vi "async stream processor.vi"(8 "error return queue":refnum<queue>, 9 "dataset RID":string, 10 "api key":string, 11 "data queue":refnum<queue>) -> (0 "last error":errorcluster)   [LabVIEW 2020, in "Nominal-Streamer.lvlib" / "Nominal-Streamer.lvclass"]
uses:
  Nominal-Streamer.lvclass
  <vilib>/Nominal/Nominal IO Client/submodules/nominal-streaming-labview-ffi/lv_src/Channel/Channel.lvclass
  <vilib>/Nominal/Nominal IO Client/lv_src/Nominal Client/Nominal Client.lvclass/Nominal Client.ctl
  <vilib>/Nominal/Nominal IO Client/lv_src/User/User.lvclass
  <vilib>/Nominal/Nominal IO Client/lv_src/Nominal Client/Nominal Client.lvclass
  <vilib>/Nominal/Nominal IO Client/lv_src/nominal types/workspace/workspace.lvclass
  <vilib>/Nominal/Nominal IO Client/submodules/reqwest-labview/lv-src/reqwest/reqwest.lvclass
  Nominal-Streamer.lvclass/Nominal-Streamer.ctl
  86105a90-7170-41be-9865-40c2d640c79f.vi
  <vilib>/Nominal/Nominal IO Client/submodules/nominal-streaming-labview-ffi/lv_src/Stream/Stream.lvclass
  <vilib>/Nominal/Nominal IO Client/lv_src/datasources/dataset/dataset.lvclass
  <vilib>/Utility/miscctls.llb/LVMapReplaceAction.ctl
  <vilib>/Utility/SystemLogging/NI_SystemLogging.lvlib
  async queue data.ctl
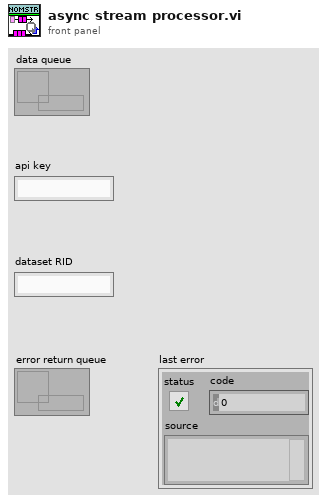
[diagram p1: front panel]
types:
  T1 = typedef "LVMapReplaceAction.ctl" = enum32{"Modify Entry only if found", "Add or Modify Entry", "Delete Entry"}
  T2 = typedef "Nominal-Streamer.lvlib/Nominal-Streamer.lvclass/async queue data.ctl" = cluster{"data values":waveform(dbl)[], "data names":string[]}
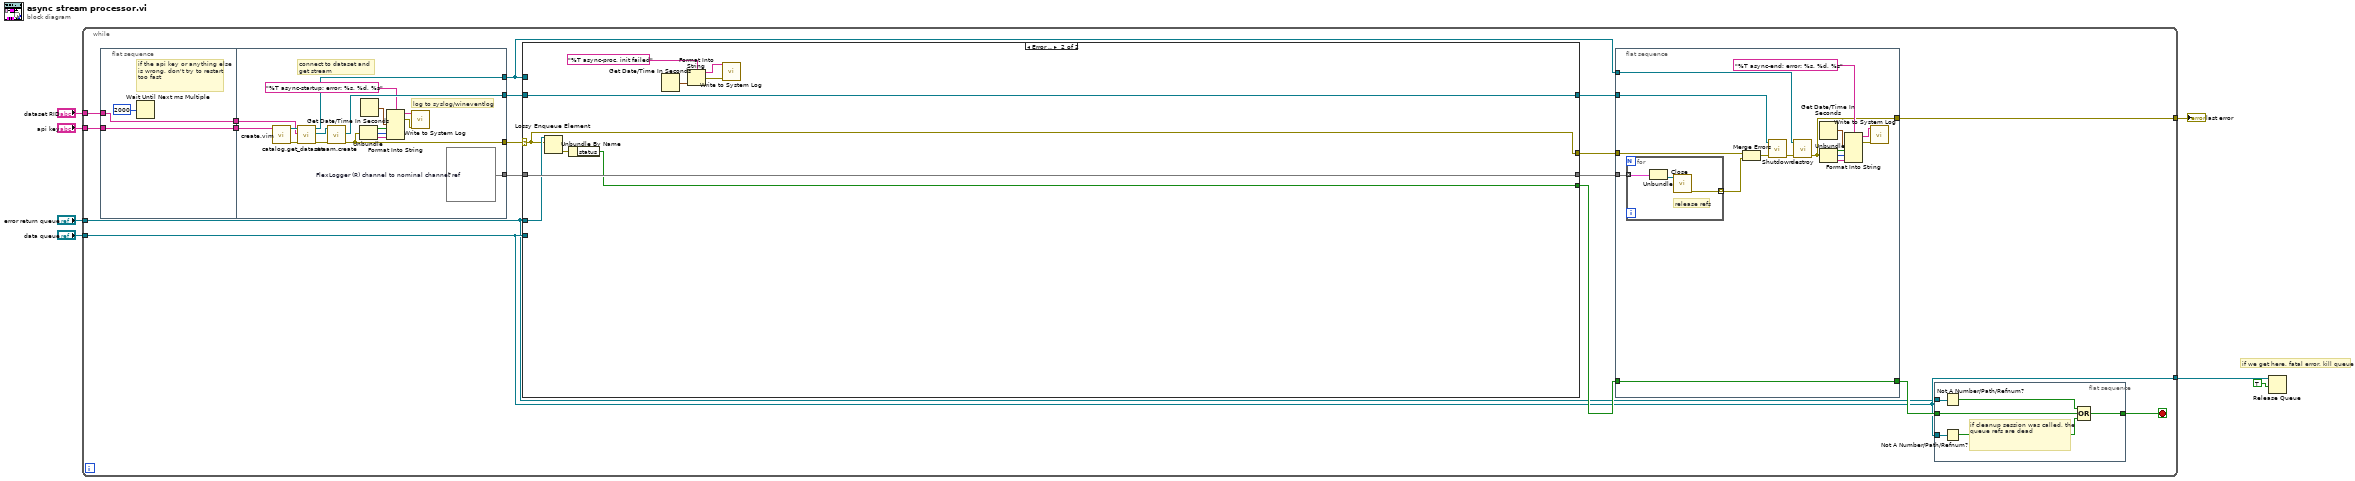
[diagram p0: block diagram]
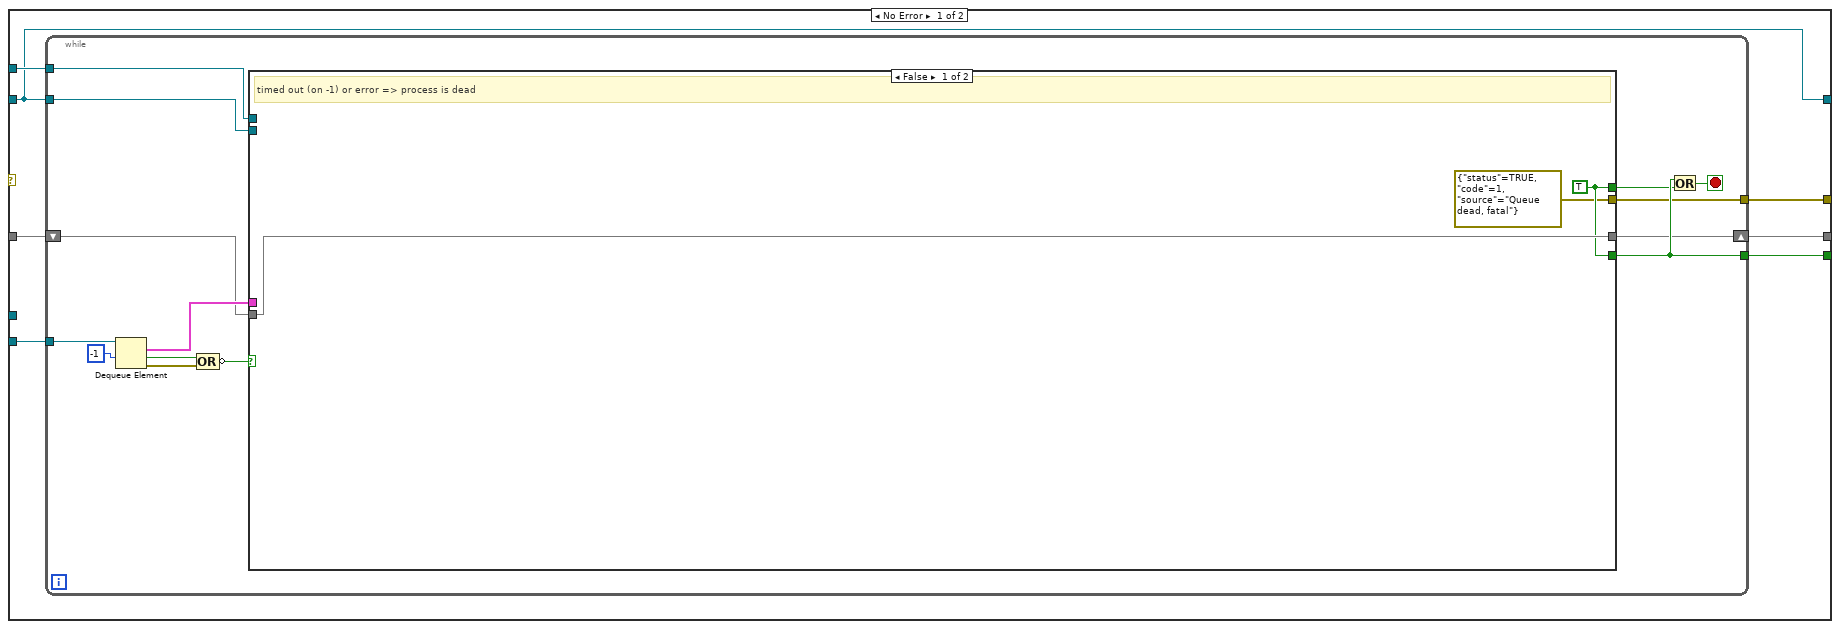
[diagram p2: hidden frame]
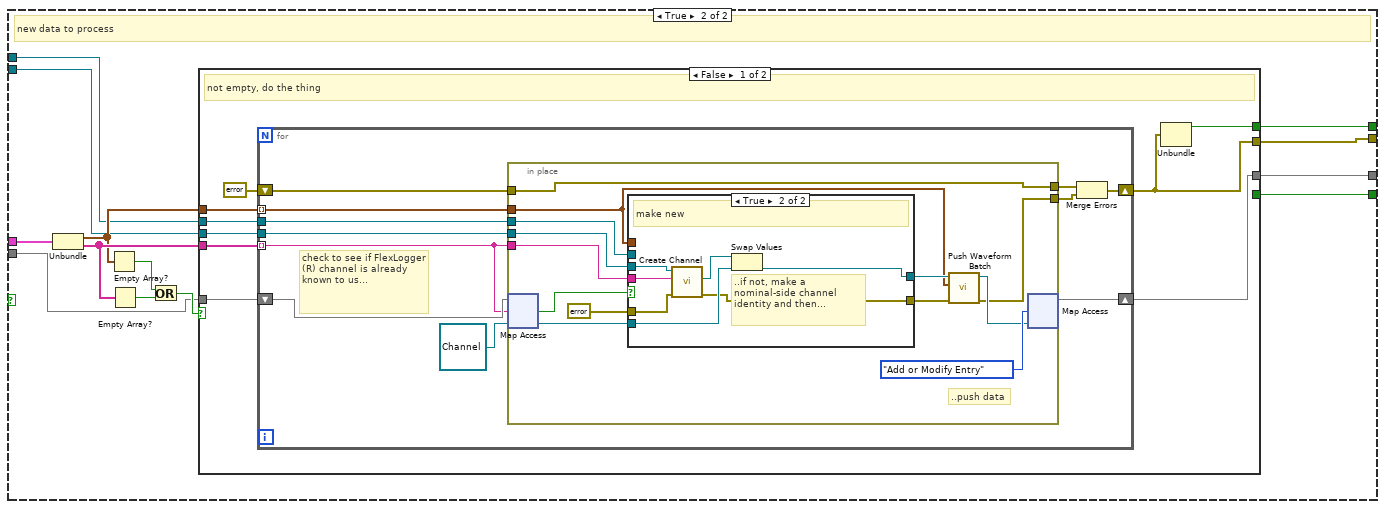
[diagram p3: hidden frame]
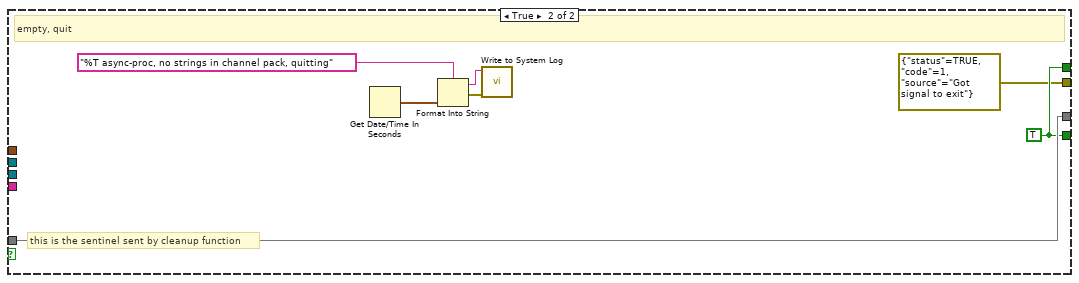
[diagram p5: hidden frame]
diagram:
  # "if we get here, fatal error, kill queue"
  n1 = while {
    tunnel: "data queue" -> [w9]
    tunnel: "api key" -> [w23]
    tunnel: "dataset RID" -> [w22]
    tunnel: [w9] -> w4
    tunnel: [w11] -> w2
    tunnel: "error return queue" -> [w8]
    stop <- w10 stop-if-true
    n2 = flat-sequence {
      tunnel: w22 -> [w128]
      tunnel: w23 -> [w129]
      tunnel: [w129] -> w16
      tunnel: [w128] -> w15
      tunnel: [w140] -> w21
      tunnel: [w133] -> w18
      tunnel: w16 -> [w146]
      tunnel: w15 -> [w144]
      tunnel: [w139] -> w14
      tunnel: [w138] -> w13
      frame #0 {
        # "if the api key or anything else is wrong, don't try to restart too fast"
        n3 = Wait Until Next ms Multiple(millisecond multiple=u32 2000) -> ()  [unwired: 1 out]
      }
      frame #1 {
        w140 = map{string, refnum<class "Channel.lvclass">} {}  # FlexLogger (R) channel to nominal channel ref
        # "connect to dataset and get stream"
        # "log to syslog/wineventlog"
        n4 = call "create.vim"("API Token (string or path)"=w146) -> ("error out"=w143:errorcluster, "Nominal Client"=w145:refnum<class "Nominal Client.lvclass">)  [unwired: 8 in, 1 out]
        n5 = call <vilib>:"catalog.get_dataset.vi"("error in"=w143, "Dataset RID"=w144, "Nominal Client in"=w145) -> ("error out"=w141:errorcluster, "Dataset"=w142:refnum<class "dataset.lvclass">, "Nominal Client out"=w139:refnum<class "Nominal Client.lvclass">)  [unwired: 6 in]
        n6 = call <vilib>:"stream.create.vi"("error in (no error)"=w141, "dataset in"=w142) -> ("error out"=w133:errorcluster, "Stream"=w138:refnum<class "Stream.lvclass">)  [unwired: 7 in, 1 out]
        n7 = Unbundle(w133) -> ("status"=w132:bool, "code"=w131:i32, "source"=w130:string)
        n8 = Get Date/Time In Seconds() -> (seconds since 1Jan1904=w136:timestamp)
        n9 = Format Into String(format string="%T async-startup; error: %s, %d, %s", w136, w132, w131, w130) -> (resulting string=w135:string, error out=w137:errorcluster)  [unwired: 2 in]
        n10 = call <vilib>:"Write to System Log.vi"("error in (no error)"=w137, "message"=w135) -> ()  [unwired: 9 in, 1 out]
      }
    }
    n11 = case shown="Error .." w18 {
      selector: w18 -> [_ w123]
      tunnel: w9 -> [w37 _]
      tunnel: [w36 w121] -> w24
      tunnel: w21 -> [w35 w126]
      tunnel: [w34 w126] -> w20
      tunnel: [w33 w123] -> w17
      tunnel: w14 -> [w32 _]
      tunnel: w13 -> [w31 w125]
      tunnel: [w31 w125] -> w12
      tunnel: w8 -> [_ w124]
      frame No Error {
        n12 = while {
          tunnel: w37 -> [w51]
          tunnel: [w45] -> w36
          shift-right: [w44] -> w34
          shift-left: w35 -> [w43]
          tunnel: [w40] -> w33
          tunnel: w32 -> [w39]
          tunnel: w31 -> [w38]
          stop <- w42 stop-if-true
          n13 = Dequeue Element(queue=w51, timeout in ms (-1)=-1) -> (element=w46:T2, timed out?=w49:bool, error out=w48:errorcluster)  [unwired: 1 in, 1 out]
          n14 = Compound Arithmetic op=OR(w49, w48) -> (invert w47:bool)
          n15 = case shown="False" w47 {
            tunnel: w46 -> [_ w67]
            tunnel: [w53 w63] -> w45
            tunnel: [w54 w62] -> w44
            tunnel: w43 -> [w54 w61]
            tunnel: [w53 w60] -> w41
            tunnel: [errorcluster {"status"=TRUE, "code"=1, "source"="Queue dead, fatal"} ("error in (no error)") w57] -> w40
            tunnel: w39 -> [_ w56]
            tunnel: w38 -> [_ w55]
            frame False {
              w53 = TRUE
              # "timed out (on -1) or error => process is dead"
            }
            frame True {
              # "new data to process"
              n16 = Unbundle(w67) -> ("data values"=w58:waveform(dbl)[], "data names"=w59:string[])
              n17 = Empty Array?(array=w58) -> (empty?=w65:bool)
              n18 = Empty Array?(array=w59) -> (empty?=w66:bool)
              n19 = Or(x=w65, y=w66) -> (x .or. y?=w64:bool)
              n20 = case shown="False" w64 {
                tunnel: [_ w115] -> w63
                tunnel: [w75 w116] -> w62
                tunnel: w61 -> [w76 w116]
                tunnel: [w70 w115] -> w60
                tunnel: w59 -> [w74 _]
                tunnel: w58 -> [w73 _]
                tunnel: [w71 errorcluster {"status"=TRUE, "code"=1, "source"="Got signal to exit"} ("error in (no error)")] -> w57
                tunnel: w56 -> [w69 _]
                tunnel: w55 -> [w68 _]
                frame False {
                  # "not empty, do the thing"
                  n21 = for {
                    shift-right: [w86] -> w75
                    shift-left: w76 -> [w87]
                    tunnel: w74 -> [w79] mode=indexing
                    tunnel: w73 -> [w83] mode=indexing
                    shift-right: [w78] -> w71
                    shift-left: errorcluster {"status"=FALSE, "code"=0, "source"=""} ("error in (no error)") -> [w85]
                    tunnel: w69 -> [w82]
                    tunnel: w68 -> [w81]
                    # "check to see if FlexLogger (R) channel is already known to us..."
                    n22 = in-place {
                      in-place-border: w85 -> [w88]
                      in-place-border: [w94] -> w84
                      in-place-border: w83 -> [w93]
                      in-place-border: w82 -> [w92]
                      in-place-border: w81 -> [w91]
                      in-place-border: w79 -> [w90]
                      in-place-border: [w88] -> w77
                      # "..push data"
                      n23 = in-place-map #1(w87, w79, refnum<class "Channel.lvclass"> refnum ("Channel")) -> (w96:refnum<class "Channel.lvclass">, w99:bool)
                      n24 = case shown="True" w99 {
                        tunnel: errorcluster {"status"=FALSE, "code"=0, "source"=""} ("error in (no error)") -> [w102 w104]
                        tunnel: [w102 w103] -> w95
                        tunnel: [w101 w106] -> w97
                        tunnel: w96 -> [w101 w107]
                        tunnel: w93 -> [_ _]
                        tunnel: w92 -> [_ _]
                        tunnel: w91 -> [_ w109]
                        tunnel: w90 -> [_ w105]
                        frame False {
                          # "...if so, do nada then..."
                          # "extant"
                        }
                        frame True {
                          # "..if not, make a nominal-side channel identity and then..."
                          # "make new"
                          n25 = call <vilib>:"Create Channel.vi"("error in (no error)"=w104, "Channel Name"=w105, "Nominal Streaming in"=w109) -> ("error out"=w103:errorcluster, "Channel"=w108:refnum<class "Channel.lvclass">)  [unwired: 6 in, 1 out]
                          n26 = Swap Values(12:w108, 14:w107) -> (3:w106:refnum<class "Channel.lvclass">)  [unwired: 1 in, 1 out]
                        }
                      }
                      n27 = call <vilib>:"Push Waveform Batch.vi"("error in (no error)"=w95, "Waveform"=w93, "Channel in"=w97) -> ("error out"=w94:errorcluster, "Channel out"=w98:refnum<class "Channel.lvclass">)  [unwired: 7 in]
                      n28 = in-place-map #1(w98, LVMapReplaceAction."Add or Modify Entry" ("action")) -> (w86:map{string, refnum<class "Channel.lvclass">})  [unwired: 2 out]
                    }
                    n29 = Merge Errors(w77, w84) -> (w78:errorcluster)
                  }
                  n30 = Unbundle(w71) -> ("status"=w70:bool)  [unwired: 2 out]
                }
                frame True {
                  w115 = TRUE
                  # "this is the sentinel sent by cleanup function"
                  # "empty, quit"
                  n31 = Get Date/Time In Seconds() -> (seconds since 1Jan1904=w112:timestamp)
                  n32 = Format Into String(format string="%T async-proc, no strings in channel pack, quitting", w112) -> (resulting string=w111:string, error out=w113:errorcluster)  [unwired: 2 in]
                  n33 = call <vilib>:"Write to System Log.vi"("error in (no error)"=w113, "message"=w111) -> ()  [unwired: 9 in, 1 out]
                }
              }
            }
          }
          n34 = Or(x=w45, y=w41) -> (x .or. y?=w42:bool)
        }
      }
      frame Error {
        n35 = Lossy Enqueue Element(queue=w124, element=w123) -> (error out=w122:errorcluster)  [unwired: 1 in, 3 out]
        n36 = Unbundle By Name(w122) -> ("status"=w121:bool)
        n37 = Get Date/Time In Seconds() -> (seconds since 1Jan1904=w119:timestamp)
        n38 = Format Into String(format string="%T async-proc, init failed", w119) -> (resulting string=w118:string, error out=w120:errorcluster)  [unwired: 2 in]
        n39 = call <vilib>:"Write to System Log.vi"("error in (no error)"=w120, "message"=w118) -> ()  [unwired: 9 in, 1 out]
      }
    }
    n40 = flat-sequence {
      tunnel: w24 -> [w162]
      tunnel: w20 -> [w158]
      tunnel: [w162] -> w19
      tunnel: w17 -> [w155]
      tunnel: w14 -> [w161]
      tunnel: w12 -> [w159]
      tunnel: [w147] -> w11
      frame #0 {
        n41 = for {
          tunnel: w158 -> [w165] mode=indexing
          tunnel: [w163] -> w157 mode=indexing
          # "release refs"
          n42 = Unbundle(w165) -> ("Channel"=w164:refnum<class "Channel.lvclass">)  [unwired: 1 out]
          n43 = call <vilib>:"Close.vi"("Channel in"=w164) -> ("error out"=w163:errorcluster)  [unwired: 10 in]
        }
        n44 = Merge Errors(w155, w157) -> (w156:errorcluster)
        n45 = call <vilib>:"Shutdown.vi"("error in (no error)"=w156, "Nominal Streaming in"=w159) -> ("error out"=w160:errorcluster)  [unwired: 8 in, 1 out]
        n46 = call <vilib>:"destroy.vi"("error in"=w160, "Nominal Client"=w161) -> ("error out"=w147:errorcluster)  [unwired: 9 in]
        n47 = Get Date/Time In Seconds() -> (seconds since 1Jan1904=w153:timestamp)
        n48 = Unbundle(w147) -> ("status"=w150:bool, "code"=w149:i32, "source"=w148:string)
        n49 = Format Into String(format string="%T async-end; error: %s, %d, %s", w153, w150, w149, w148) -> (resulting string=w152:string, error out=w154:errorcluster)  [unwired: 2 in]
        n50 = call <vilib>:"Write to System Log.vi"("error in (no error)"=w154, "message"=w152) -> ()  [unwired: 9 in, 1 out]
      }
    }
    n51 = flat-sequence {
      tunnel: w19 -> [w30]
      tunnel: [w29] -> w10
      tunnel: w9 -> [w26]
      tunnel: w8 -> [w25]
      frame #0 {
        # "if cleanup session was called, the queue refs are dead"
        n52 = Not A Number/Path/Refnum?(number/path/refnum=w25) -> (NaN/Path/Refnum?=w28:bool)
        n53 = Not A Number/Path/Refnum?(number/path/refnum=w26) -> (NaN/Path/Refnum?=w27:bool)
        n54 = Compound Arithmetic op=OR(w28, w30, w27) -> (w29:bool)
      }
    }
  }
  "last error" <- w2
  n55 = Release Queue(queue=w4, force destroy? (F)=TRUE) -> ()  [unwired: 1 in, 3 out]
